vi "Write Log File.vi"(8 "error in":errorcluster, 10 "Log File":path, 11 "File Logger in":refnum<class "File Logger.lvclass">) -> (0 "error out":errorcluster, 3 "File Logger out":refnum<class "File Logger.lvclass">)   [LabVIEW 2026, in "File Logger.lvlib" / "File Logger.lvclass"]
doc: "Data accessor."
uses:
  File Logger.lvclass
  File Logger.lvclass/File Logger.ctl
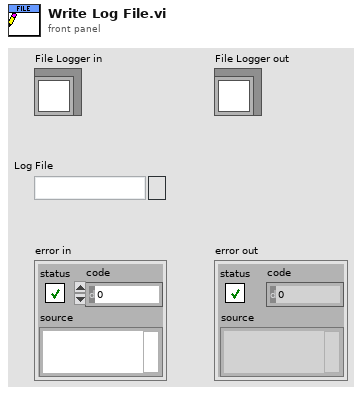
[diagram p1: front panel]
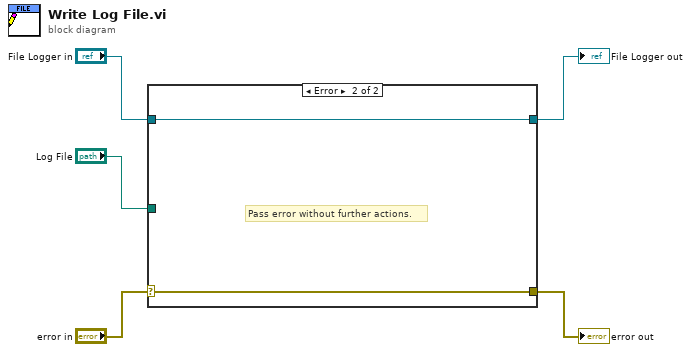
[diagram p0: block diagram]
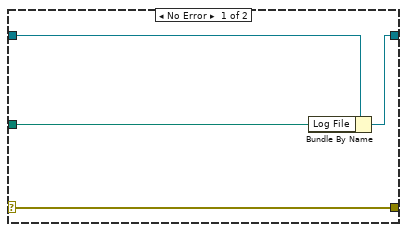
[diagram p2: hidden frame]
diagram:
  n1 = case shown="Error" "error in" {
    selector: "error in" -> [w9 w11]
    tunnel: [w9 w11] -> w4
    tunnel: [w7 w10] -> w2
    tunnel: "File Logger in" -> [w8 w10]
    tunnel: "Log File" -> [w6 _]
    frame No Error {
      n2 = Bundle By Name(cluster=w8, "Log File"=w6) -> (w7:refnum<class "File Logger.lvclass">)
    }
    frame Error {
      # "Pass error without further actions."
    }
  }
  "error out" <- w4
  "File Logger out" <- w2
